vi "tdms selection_A.vi"(6 "error in":errorcluster, 8 "string":string="tdms", 11 "Filename List":string[](array[string])) -> (0 "size(s)":i32, 3 "Array 2":string[](array[string]), 4 "error out":errorcluster)   [LabVIEW 2018]
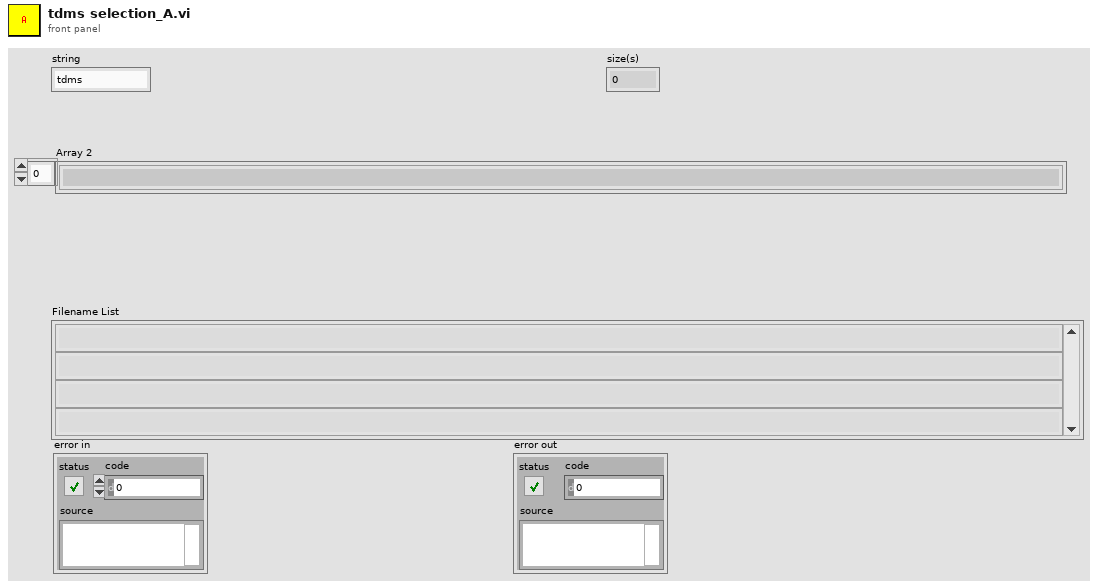
[diagram p1: front panel]
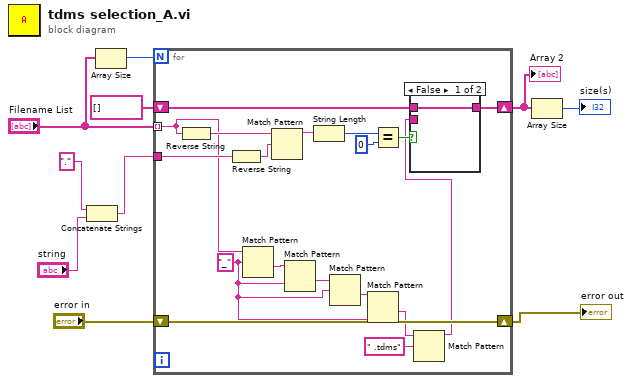
[diagram p0: block diagram]
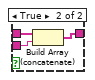
[diagram p2: hidden frame]
diagram:
  n1 = Concatenate Strings("." ("string"), "string") -> (w5:string)
  n2 = Array Size(array="Filename List") -> (size(s)=w10:i32)
  n3 = for {
    N: w10 -> [_]
    tunnel: "Filename List" -> [w18] mode=indexing
    shift-right: [w22] -> w7
    shift-left: string[] [] -> [w21]
    tunnel: w5 -> [w20]
    shift-right: [w19] -> w1
    shift-left: "error in" -> [w19]
    w14 = "_" ("regular expression")
    n4 = Reverse String(1:w18) -> (0:w28:string)
    n5 = Reverse String(1:w20) -> (0:w27:string)
    n6 = Match Pattern(string=w18, regular expression=w14) -> (after substring=w17:string)  [unwired: 1 in, 3 out]
    n7 = Match Pattern(string=w28, regular expression=w27) -> (before substring=w26:string)  [unwired: 1 in, 3 out]
    n8 = Match Pattern(string=w17, regular expression=w14) -> (after substring=w16:string)  [unwired: 1 in, 3 out]
    n9 = String Length(string=w26) -> (length=w25:i32)
    n10 = Match Pattern(string=w16, regular expression=w14) -> (after substring=w15:string)  [unwired: 1 in, 3 out]
    n11 = Match Pattern(string=w15, regular expression=w14) -> (after substring=w13:string)  [unwired: 1 in, 3 out]
    n12 = Equal?(x=w25, y=0) -> (x = y?=w23:bool)
    n13 = Match Pattern(string=w13, regular expression=" .tdms") -> (before substring=w11:string)  [unwired: 1 in, 3 out]
    n14 = case shown="False" w23 {
      tunnel: w11 -> [_ w32]
      tunnel: [w29 w31] -> w22
      tunnel: w21 -> [w29 w30]
      frame False {
      }
      frame True {
        n15 = Build Array (concatenate)(w30, w32) -> (w31:string[])
      }
    }
  }
  "Array 2" <- w7
  "error out" <- w1
  n16 = Array Size(array=w7) -> (size(s)=→"size(s)":i32)
